vi "Analyze Error Data_LV2014.vi"() -> ()   [LabVIEW 2014]
panel:
  in  "String":string
  out ">=1 bad signals per fiber":bool[](array[boolean])
  out "number of bad signals per fiber":i32[](array[numeric])
  out "Signal quality insufficient (all channels)":bool[][](array[boolean])
  # "Shows how to analyze the answer of the \"e?> command"
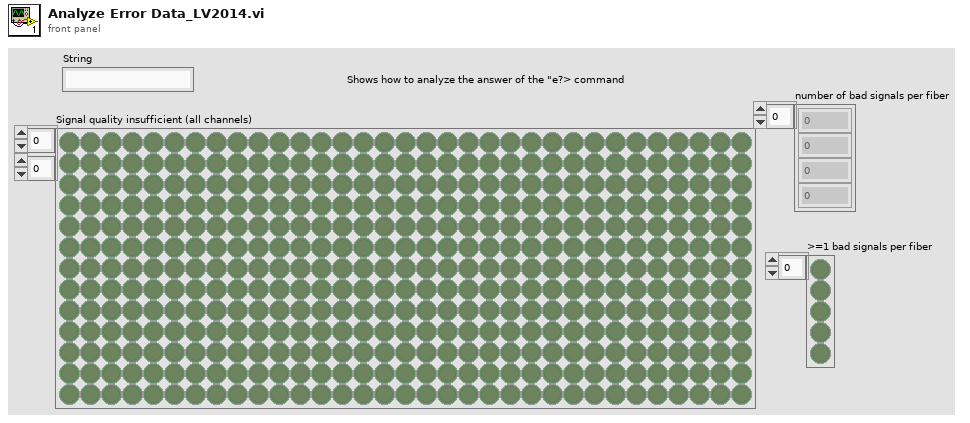
[diagram p1: front panel]
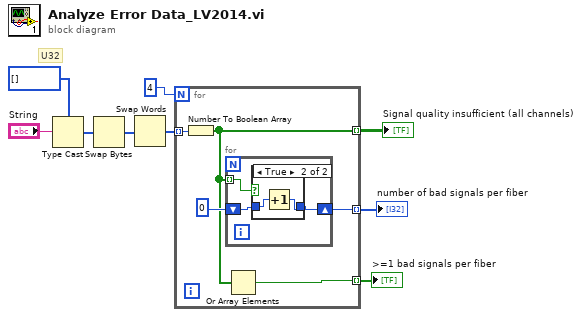
[diagram p0: block diagram]
diagram:
  # "U32"
  n1 = Type Cast(type=u32[] [] ("Angehängtes Array"), x="String") -> (*(type *) &x=w9:u32[])
  n2 = Swap Bytes ("Bytes tauschen")(anything=w9) -> (byte swapped=w8:u32[])
  n3 = Swap Words ("Words tauschen")(1:w8) -> (0:w6:u32[])
  n4 = for {
    N: 4 -> [_]
    tunnel: w6 -> [w14] mode=indexing
    tunnel: [w11] -> w5 mode=indexing
    tunnel: [w12] -> w4 mode=indexing
    tunnel: [w10] -> w2 mode=indexing
    n5 = Number To Boolean Array ("Zahl nach boolesches Array")(number=w14) -> (Boolean array=w11:bool[])
    n6 = for {
      tunnel: w11 -> [w15] mode=indexing
      shift-right: [w16] -> w12
      shift-left: 0 -> [w17]
      n7 = case shown="True" w15 {
        tunnel: w17 -> [w18 w20]
        tunnel: [w18 w19] -> w16
        frame False {
        }
        frame True {
          n8 = Increment(x=w20) -> (x+1=w19:i32)
        }
      }
    }
    n9 = Or Array Elements ("ODER (Array-Elemente)")(Boolean array=w11) -> (logical OR=w10:bool)
  }
  "Signal quality insufficient (all channels)" <- w5
  "number of bad signals per fiber" <- w4
  ">=1 bad signals per fiber" <- w2
